vi "Pose3d_Log.vi"(9 "end Pose3d":T2={"Translation3d"={"X"=0.0, "Y"=0.0, "Z"=0.0}, "Rotation3d"={"Q_quaternion"={"R"=1.0, "V"=[0.0, 0.0, 0.0]}}} {"Translation3d"."Z" format="%14.3f"; "Translation3d"."Y" format="%14.3f"; "Translation3d"."X" format="%14.3f"}, 11 "in Pose3d":T2={"Translation3d"={"X"=0.0, "Y"=0.0, "Z"=0.0}, "Rotation3d"={"Q_quaternion"={"R"=1.0, "V"=[0.0, 0.0, 0.0]}}} {"Translation3d"."Z" format="%14.3f"; "Translation3d"."Y" format="%14.3f"; "Translation3d"."X" format="%14.3f"}) -> (0 "Error":bool, 3 "out Twist3d":T1)   [LabVIEW 2019, in "Trajectory_Library.lvlib"]
doc: "Returns a Twist3d that maps this pose to the end pose. If c is the output of a.Log(b), then a.Exp(c) would yield b.\n \nParmeters:\n - IN POSE3D - The current POSE data structure\n - OTHER POSE3D - The end pose for the transformation.\n\nReturns:\n - OUT TWIST3D - The twist that maps this to end.\n - Error -- boolean -- If value is TRUE, an error occured."
uses:
  Trajectory_Library.lvlib
  TypeDef/POSE3D.ctl
  TypeDef/TRANSLATION3D.ctl
  TypeDef/ROTATION3D.ctl
  TypeDef/QUATERNION.ctl
  TypeDef/TWIST3D.ctl
  <vilib>/Analysis/baseanly.llb/Real A x B.vi
  Pose3d_New_Trans3dRot3d.vi
  Transform3d_Create_Pose3dPose3d.vi
  Transform3d_GetRotation3d.vi
  Transform3d_GetTranslation3d.vi
  MatBuilder_Fill.vi
  Pose3d_getTranslation3d.vi
  Translation3d_GetXYZ.vi
  MatBuilder_Create.vi
  Quaternion_Get_Vect.vi
  Quaternion_Get_W.vi
  <vilib>/Analysis/7linalg.llb/Matrix Power.vi
  <vilib>/Analysis/7linalg.llb/Real Matrix Power.vi
  <vilib>/Analysis/7linalg.llb/Matrix Exp.vi
  <vilib>/Analysis/7linalg.llb/Real Matrix Exp.vi
  Transform3d_Create_Trans3dRot3d.vi
  Translation3d_Minus.vi
  Translation3d_RotateBy.vi
  Rotation3d_UnaryMinus.vi
  Rotation3d_Minus.vi
  Translation3d_Create.vi
  Quaternion_New.vi
  Quaternion_Times.vi
  Quaternion_Inverse.vi
  Quaternion_Get_All.vi
  Rotation3d_Create_Quaternion.vi
  Rotation3d_RotateBy.vi
  Quaternion_Normalize.vi
  Quaternion_New_Default.vi
  <vilib>/Analysis/7linalg.llb/Create Special Matrix.vi
  <vilib>/Analysis/7linalg.llb/Create Special Real Matrix.vi
  <vilib>/Analysis/Matrix/Numeric/Conversions/Array To Matrix.vi
  <vilib>/Analysis/Matrix/Numeric/Conversions/Array To Matrix - RA.vi
  <vilib>/Analysis/7linalg.llb/Matrix Logarithm.vi
  <vilib>/Analysis/7linalg.llb/Real Matrix Logarithm.vi
  <vilib>/Analysis/Matrix/Numeric/Complex/Complex To Cartesian.vi
  <vilib>/Analysis/Matrix/Numeric/Complex/Complex To Cartesian - CM.vi
  <vilib>/Analysis/Matrix/Numeric/Multiply/Multiply - RM,R.vi
  <vilib>/Analysis/Matrix/Numeric/Subtract/Subtract - RM,RM.vi
  <vilib>/Analysis/Matrix/Numeric/Add/Add - RM,RM.vi
  <vilib>/Analysis/Matrix/NI_Matrix.lvlib
  <vilib>/Analysis/NI_AALBase.lvlib
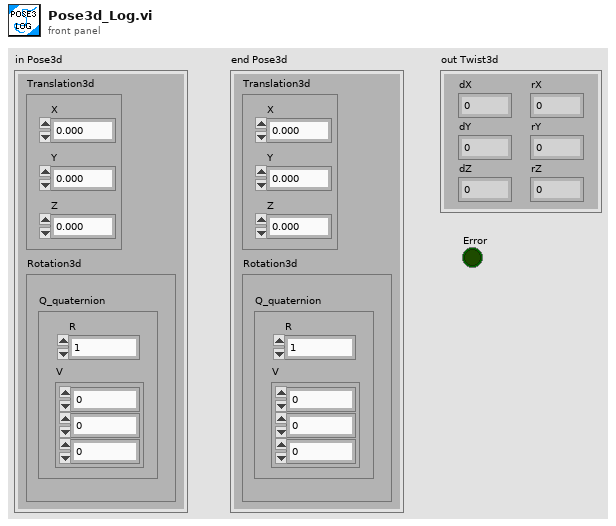
[diagram p1: front panel]
types:
  T1 = typedef "Trajectory_Library.lvlib/TWIST3D.ctl" = cluster{"dX":dbl, "dY":dbl, "dZ":dbl, "rX":dbl, "rY":dbl, "rZ":dbl}
  T2 = typedef "Trajectory_Library.lvlib/POSE3D.ctl" = cluster{"Translation3d":T3, "Rotation3d":T4}
  T3 = typedef "Trajectory_Library.lvlib/TRANSLATION3D.ctl" = cluster{"X":dbl, "Y":dbl, "Z":dbl}
  T4 = typedef "Trajectory_Library.lvlib/ROTATION3D.ctl" = cluster{"Q_quaternion":T5}
  T5 = typedef "Trajectory_Library.lvlib/QUATERNION.ctl" = cluster{"R":dbl, "V":dbl[]}
  T6 = typedef "NI_Matrix.lvlib/RealMatrix.ctl" = dbl[][]
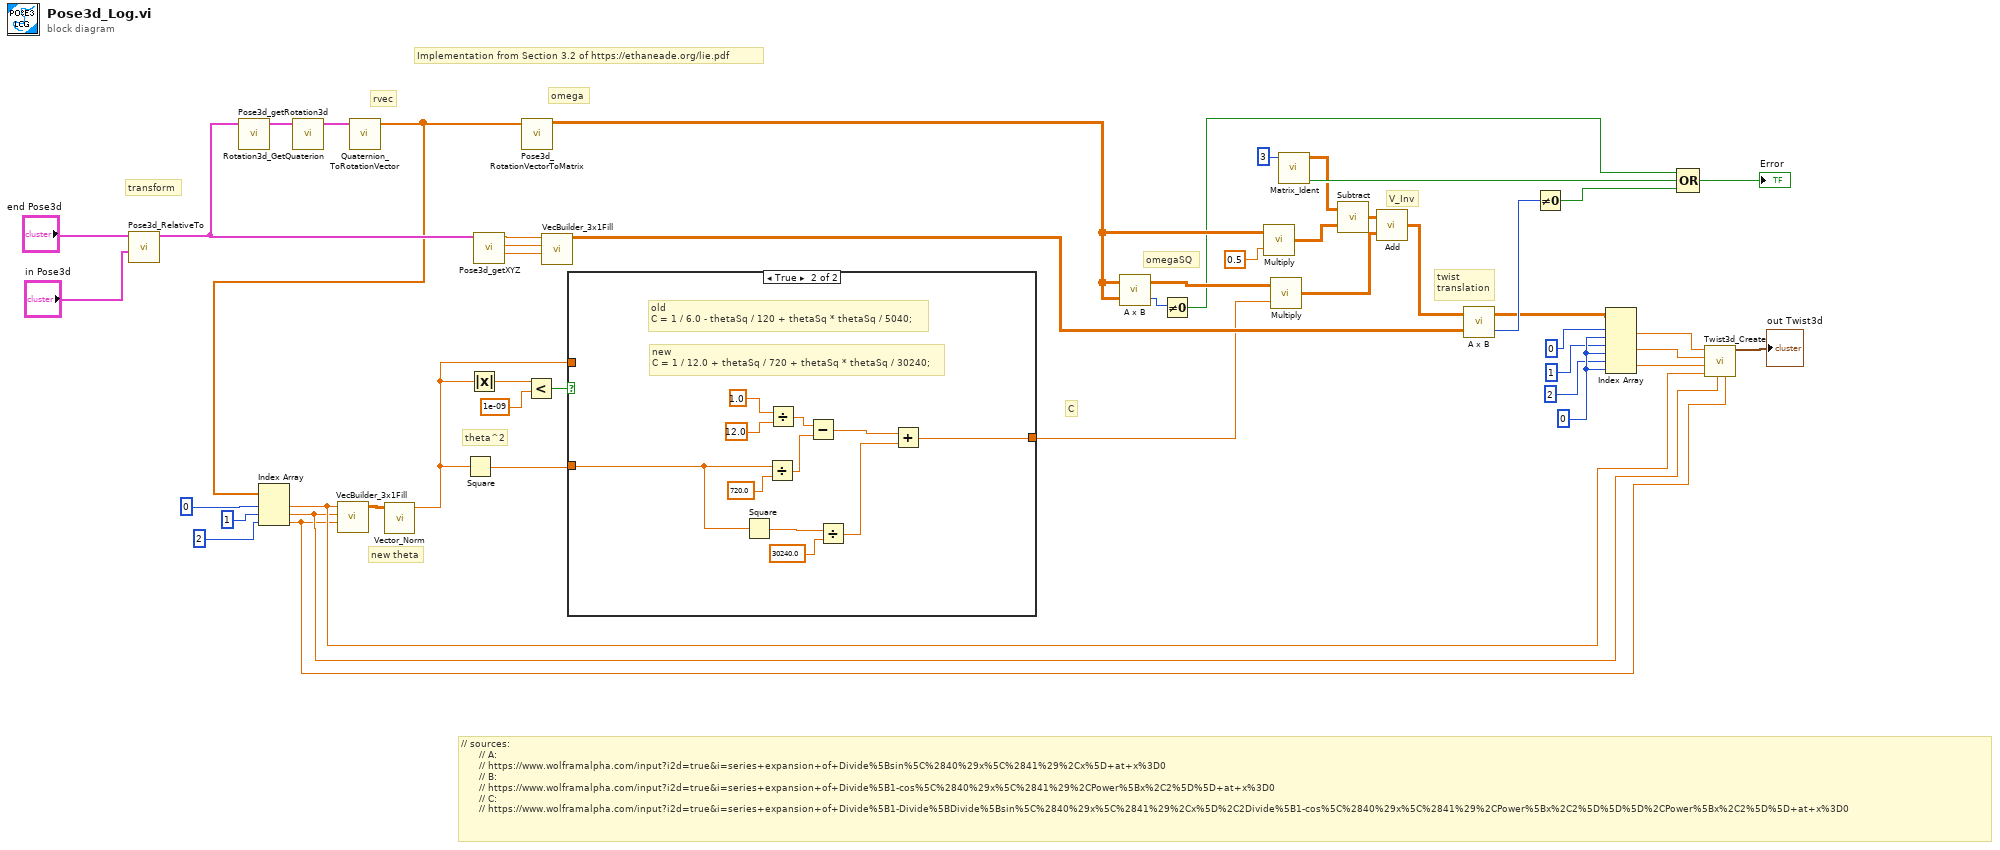
[diagram p0: block diagram]
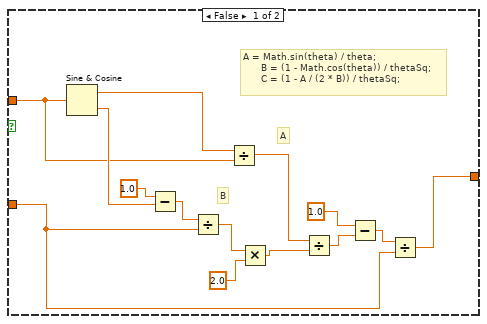
[diagram p2: hidden frame]
diagram:
  w37 = 0 ("index (col)")
  # "// sources:\n      // A:\n      // https://www.wolframalpha.com/input?i2d=true&i=series+expansion+of+Divide%5Bsin%5C%2840%29x%5C%2841%29%2Cx%5D+at+x%3D0\n      // B:\n      // https://www.wolframalpha.com/input?i2d=true&i=series+expansion+of+Divide%5B1-cos%5C%2840%29x%5C%2841%29%2CPower%5Bx%2C2%5D%5D+at+x%3D0\n      // C:\n      // https://www.wolframalpha.com/input?i2d=true&i=series+expansion+of+Divide%5B1-Divide%5BDivide%5Bsin%5C%2840%29x%5C%2841%29%2Cx%5D%2C2Divide%5B1-cos%5C%2840%29x%5C%2841%29%2CPower%5Bx%2C2%5D%5D%5D%2CPower%5Bx%2C2%5D%5D+at+x%3D0"
  # "new theta"
  # "twist\ntranslation"
  # "V_Inv"
  # "omegaSQ"
  # "C"
  # "rvec"
  # "Implementation from Section 3.2 of https://ethaneade.org/lie.pdf"
  # "transform"
  # "theta^2"
  # "omega"
  n1 = call "Pose3d_RelativeTo.vi"("other Pose3d"="in Pose3d", "in Pose3d"="end Pose3d") -> ("out Pose3d"=w42:T2)  [unwired: 9 in]
  n2 = call "Pose3d_getRotation3d.vi"("in Pose3d"=w42) -> ("out Rotation3d"=w31:T4)  [unwired: 10 in]
  n3 = call "Rotation3d_GetQuaterion.vi"("in Rotation3d"=w31) -> ("out Quaterion"=w43:T5)  [unwired: 10 in]
  n4 = call "Quaternion_ToRotationVector.vi"("Quaternion"=w43) -> ("RotationVector"=w13:dbl[])  [unwired: 10 in]
  n5 = Index Array(array=w13, index #1=0 ("index"), index #2=1 ("index"), index #3=2 ("index")) -> (element #1=w7:dbl, element #2=w6:dbl, element #3=w5:dbl)
  n6 = call "VecBuilder_3x1Fill.vi"("R2"=w5, "R1"=w6, "R0"=w7) -> ("output matrix"=w9:T6)  [unwired: 8 in]
  n7 = call "Vector_Norm.vi"("Input Vector"=w9) -> ("norm"=w8:dbl)  [unwired: 10 in]
  n8 = Square(x=w8) -> (x^2=w29:dbl)
  n9 = Absolute Value(x=w8) -> (abs(x)=w14:dbl)
  n10 = call "Pose3d_getXYZ.vi"("in Pose3d"=w42) -> ("Z"=w39:dbl, "Y"=w40:dbl, "X"=w41:dbl)  [unwired: 8 in]
  n11 = call "Pose3d_RotationVectorToMatrix.vi"("RotationVector"=w13) -> ("Rotation Matrix"=w4:T6)  [unwired: 10 in]
  n12 = Less?(x=w14, y=1e-09) -> (x < y?=w45:bool)
  n13 = call "VecBuilder_3x1Fill.vi"("R2"=w39, "R1"=w40, "R0"=w41) -> ("output matrix"=w26:T6)  [unwired: 8 in]
  n14 = case shown="True" w45 {
    tunnel: w29 -> [w49 w64]
    tunnel: [w48 w62] -> w20
    tunnel: w8 -> [w56 _]
    frame False {
      # "B"
      # "A"
      # "A = Math.sin(theta) / theta;\n      B = (1 - Math.cos(theta)) / thetaSq;\n      C = (1 - A / (2 * B)) / thetaSq;"
      n15 = Sine & Cosine(0:w56) -> (1:w60:dbl, 2:w59:dbl)
      n16 = Subtract(x=1.0, y=w59) -> (x-y=w58:dbl)
      n17 = Divide(x=w58, y=w49) -> (x/y=w52:dbl)
      n18 = Divide(x=w60, y=w56) -> (x/y=w55:dbl)
      n19 = Multiply(x=w52, y=2.0) -> (x*y=w51:dbl)
      n20 = Divide(x=w55, y=w51) -> (x/y=w54:dbl)
      n21 = Subtract(x=1.0, y=w54) -> (x-y=w50:dbl)
      n22 = Divide(x=w50, y=w49) -> (x/y=w48:dbl)
    }
    frame True {
      # "new\nC = 1 / 12.0 + thetaSq / 720 + thetaSq * thetaSq / 30240;"
      # "old\nC = 1 / 6.0 - thetaSq / 120 + thetaSq * thetaSq / 5040;"
      n23 = Square(x=w64) -> (x^2=w65:dbl)
      n24 = Divide(x=w64, y=720.0) -> (x/y=w67:dbl)
      n25 = Divide(x=1.0, y=12.0) -> (x/y=w71:dbl)
      n26 = Subtract ("Subtract.vi")(x=w71, y=w67) -> (x-y=w72:dbl)
      n27 = Divide(x=w65, y=30240.0) -> (x/y=w63:dbl)
      n28 = Add ("Add.vi")(x=w72, y=w63) -> (x+y=w62:dbl)
    }
  }
  n29 = call-poly <vilib>:"A x B.vi"("B"=w4, "A"=w4) -> ("error"=w2:i32, "A x B"=w3:T6)
  n30 = Not Equal To 0?(x=w2) -> (x != 0?=w1:bool)
  n31 = call-poly <vilib>:"Multiply.vi"("Real Scalar c"=0.5 ("y"), "Real Matrix A"=w4) -> ("A * c"=w21:T6)
  n32 = call-poly <vilib>:"Multiply.vi"("Real Scalar c"=w20, "Real Matrix A"=w3) -> ("A * c"=w18:T6)
  n33 = call "Matrix_Ident.vi"("Size"=3) -> ("Error"=w27:bool, "output matrix"=w23:T6)  [unwired: 9 in]
  n34 = call-poly <vilib>:"Subtract.vi"("Real Matrix B"=w21, "Real Matrix A"=w23) -> ("A - B"=w19:T6)
  n35 = call-poly <vilib>:"Add.vi"("Real Matrix B"=w18, "Real Matrix A"=w19) -> ("A + B"=w17:T6)
  n36 = call-poly <vilib>:"A x B.vi"("B"=w26, "A"=w17) -> ("error"=w24:i32, "A x B"=w16:T6)
  n37 = Not Equal To 0?(x=w24) -> (x != 0?=w25:bool)
  n38 = Index Array(array=w16, index (row) #1=0 ("index (row)"), index (col) #1=w37, index (row) #2=1 ("index (row)"), index (col) #2=w37, index (row) #3=2 ("index (row)"), index (col) #3=w37) -> (element #1=w34:dbl, element #2=w33:dbl, element #3=w32:dbl)
  n39 = Compound Arithmetic op=OR(w1, w27, w25) -> (→"Error":bool)
  n40 = call "Twist3d_Create.vi"("rZ"=w5, "rY"=w6, "rX"=w7, "dZ"=w32, "dY"=w33, "dX"=w34) -> ("Twist3d"=→"out Twist3d":T1)  [unwired: 5 in]
